vi "sensor mdl.vi"() -> ()   [LabVIEW 2021]
panel:
  out "x-y":dbl
  out "remaining":dbl
  in  "t":dbl
  out "Waveform Chart Z":dbl(graph)
  out "Waveform Chart X":dbl(graph)
  out "JSON data":string
  in  "Path data":path
  in  "Not stable":string
  in  "Stable":string
  out "Rotation z":dbl
  out "Driver status":string
  out "Rotation x":dbl
  out "DROWSY":bool
  out "ACTIVE":bool
  in  "stop":bool
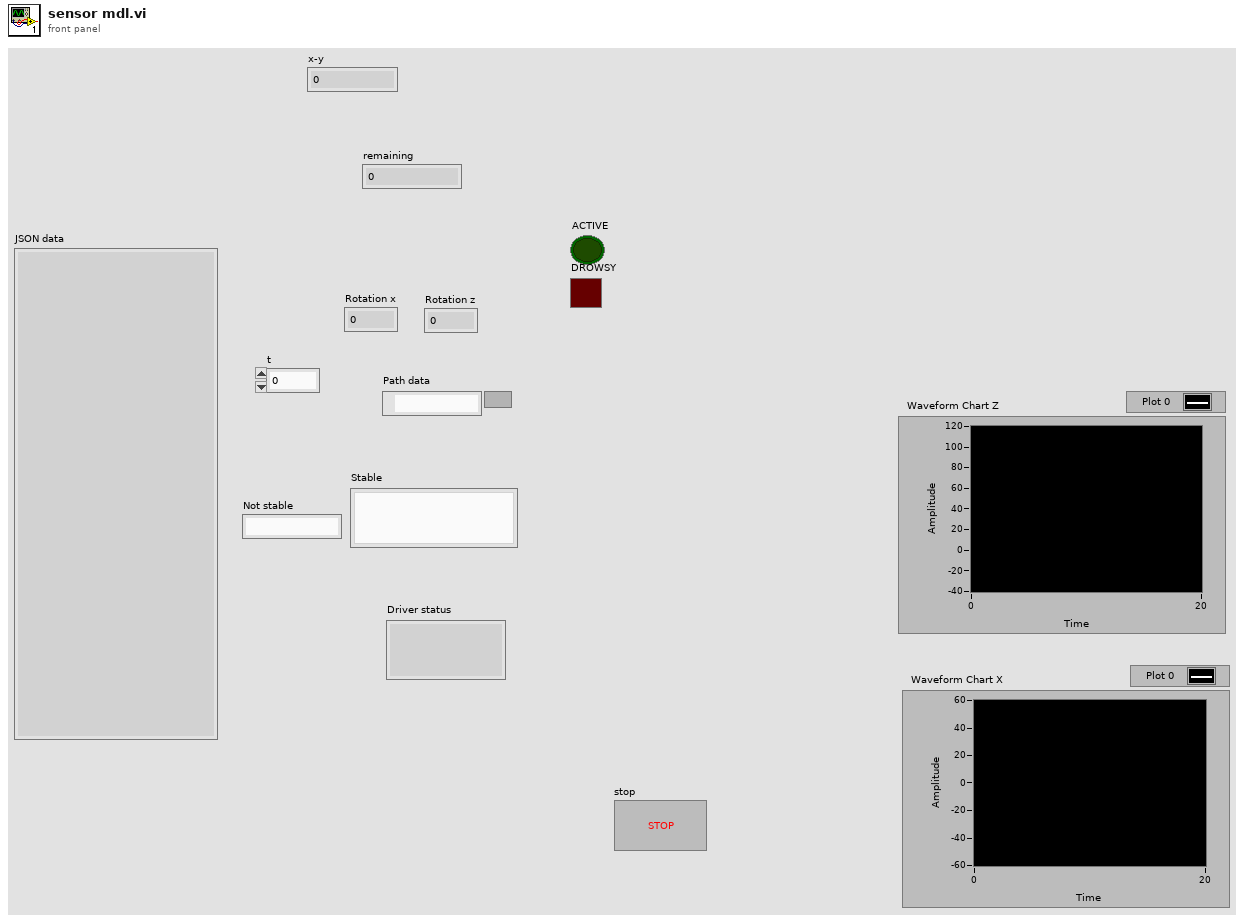
[diagram p1: front panel]
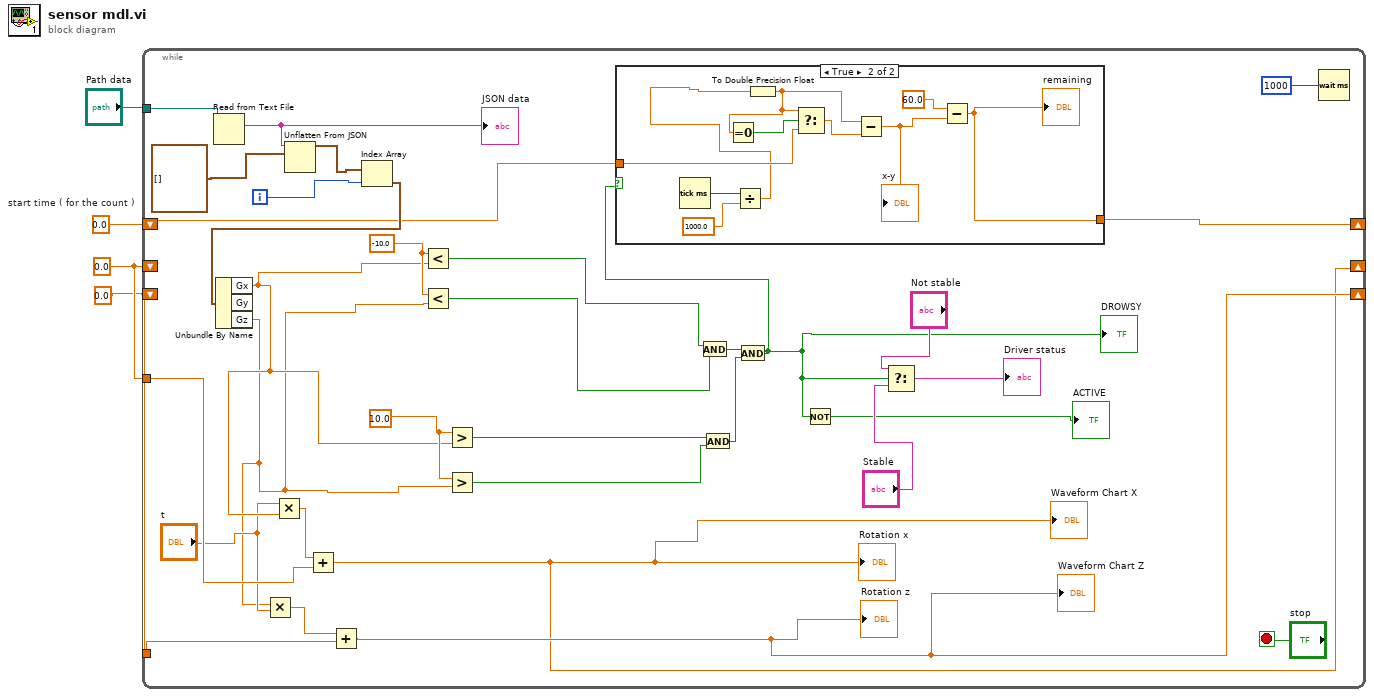
[diagram p0: block diagram]
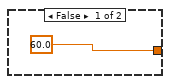
[diagram p2: hidden frame]
diagram:
  w1 = 0.0  # start time ( for the count )
  w3 = 0.0 ("y")
  w4 = 0.0 ("y")
  n1 = while {
    shift-right: [w19] -> _
    shift-left: w4 -> [_]
    tunnel: w4 -> [w33]
    shift-right: [w20] -> _
    shift-left: w3 -> [_]
    tunnel: w3 -> [w31]
    tunnel: "Path data" -> [w22]
    shift-right: [w7] -> _
    shift-left: w1 -> [w8]
    i -> [w11]
    stop <- "stop" stop-if-true
    w26 = 10.0 ("y")
    w29 = -10.0 ("y")
    n2 = Read from Text File(file (use dialog)=w22) -> (text=w13:string)  [unwired: 3 in, 3 out]
    "JSON data" <- w13
    n3 = Unflatten From JSON(JSON string=w13, type and defaults=cluster{"Gx":dbl, "Gy":dbl, "Gz":dbl}[] [] ("Array 2")) -> (value=w16:cluster{"Gx":dbl, "Gy":dbl, "Gz":dbl}[])  [unwired: 5 in, 1 out]
    n4 = Index Array(array=w16, index=w11) -> (element=w15:cluster{"Gx":dbl, "Gy":dbl, "Gz":dbl})
    n5 = Unbundle By Name(w15) -> ("Gx"=w21:dbl, "Gz"=w12:dbl)  [unwired: 1 out]
    n6 = Multiply(x=w12, y="t") -> (x*y=w30:dbl)
    n7 = Multiply(x="t", y=w21) -> (x*y=w34:dbl)
    n8 = Add(x=w34, y=w33) -> (x+y=w19:dbl)
    "Rotation x" <- w19
    "Waveform Chart X" <- w19
    n9 = Add(x=w30, y=w31) -> (x+y=w20:dbl)
    "Rotation z" <- w20
    "Waveform Chart Z" <- w20
    n10 = Less?(x=w29, y=w21) -> (x < y?=w28:bool)
    n11 = Less?(x=w29, y=w12) -> (x < y?=w27:bool)
    n12 = Greater?(x=w26, y=w21) -> (0:w25:bool)
    n13 = Greater?(x=w26, y=w12) -> (0:w24:bool)
    n14 = And(x=w28, y=w27) -> (x .and. y?=w36:bool)
    n15 = And(x=w25, y=w24) -> (x .and. y?=w35:bool)
    n16 = And(x=w36, y=w35) -> (x .and. y?=w6:bool)
    "DROWSY" <- w6
    n17 = case shown="True" w6 {
      tunnel: w8 -> [_ w43]
      tunnel: [60.0 ("start time ( for the count )") w41] -> w7
      frame False {
      }
      frame True {
        n18 = Tick Count (ms)() -> (millisecond timer value=w39:u32)
        n19 = Divide(x=w39, y=1000.0) -> (x/y=w38:dbl)
        n20 = To Double Precision Float(number=w38) -> (double precision float=w45:dbl)
        n21 = Equal To 0?(x=w45) -> (x = 0?=w44:bool)
        n22 = Select(t=w45, s=w44, f=w43) -> (s? t:f=w42:dbl)
        n23 = Subtract(x=w45, y=w42) -> (x-y=w46:dbl)
        "x-y" <- w46
        n24 = Subtract(x=60.0, y=w46) -> (x-y=w41:dbl)
        "remaining" <- w41
      }
    }
    n25 = Not(x=w6) -> (.not. x?=→"ACTIVE":bool)
    n26 = Select(t="Not stable", s=w6, f="Stable") -> (s? t:f=→"Driver status":string)
    n27 = Wait (ms)(milliseconds to wait=u32 1000) -> ()  [unwired: 1 out]
  }
